vi "虚拟计算器_六控件查看.vi"() -> ()   [LabVIEW 2023]
doc: "实验1 简易计算器设计。按课程指导书建立六个字符串显示控件、初始化、While循环及数字、运算符、等号、清除值改变事件。四则运算条件结构直接位于等号事件内。"
panel:
  in  "清除":bool
  in  "等于":bool
  in  "除":bool
  in  "乘":bool
  in  "减":bool
  in  "加":bool
  in  "小数点":bool
  in  "数字0":bool
  in  "数字9":bool
  in  "数字8":bool
  in  "数字7":bool
  in  "数字6":bool
  in  "数字5":bool
  in  "数字4":bool
  in  "数字3":bool
  in  "数字2":bool
  in  "数字1":bool
  out "运算结果":string
  out "运算符临时值":string
  out "输入2":string
  out "输入1":string
  out "输入临时值":string
  out "过程显示":string
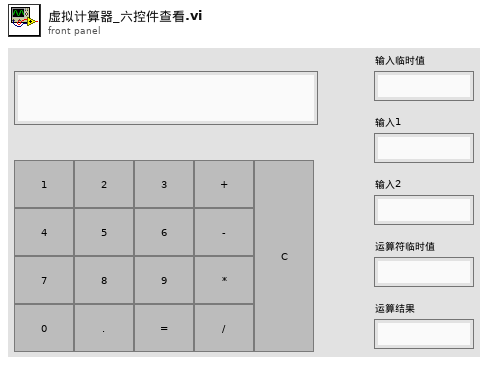
[diagram p1: front panel]
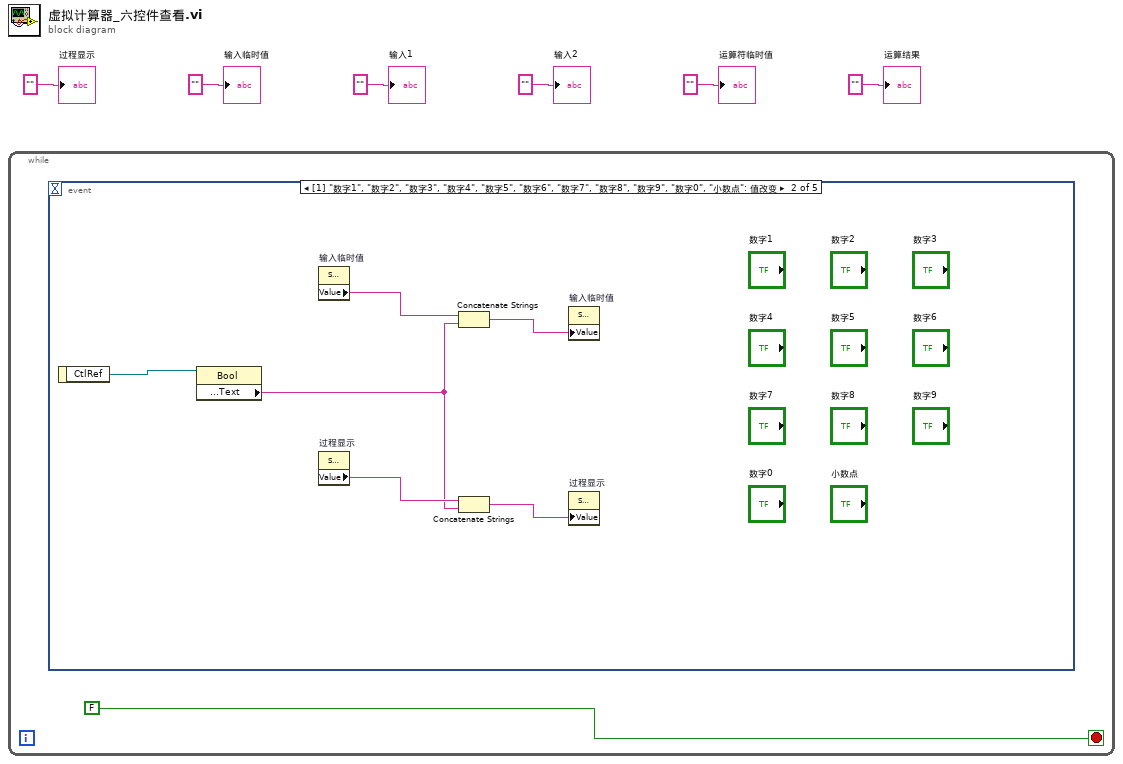
[diagram p0: block diagram]
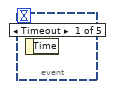
[diagram p2: hidden frame]
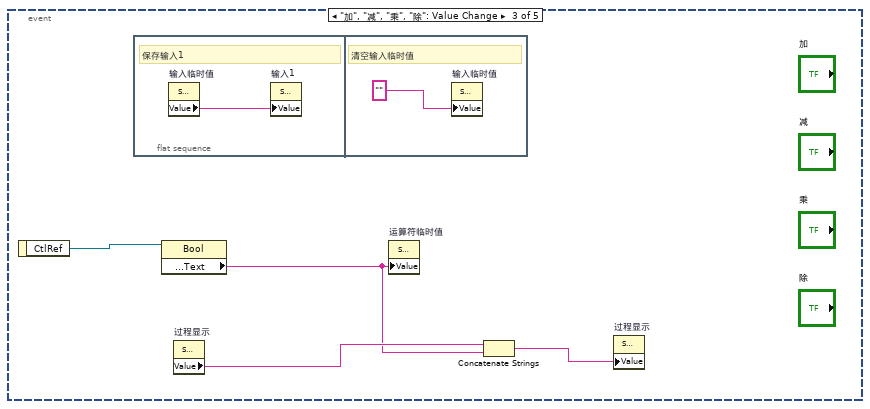
[diagram p3: hidden frame]
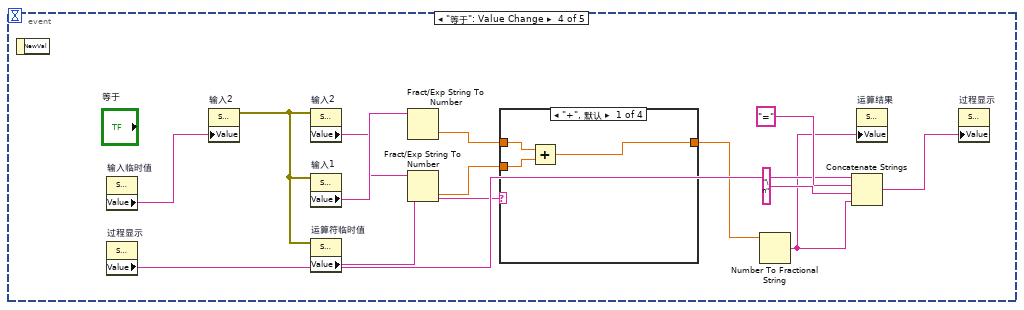
[diagram p4: hidden frame]
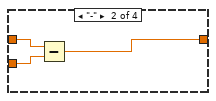
[diagram p5: hidden frame]
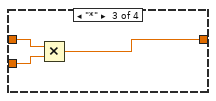
[diagram p6: hidden frame]
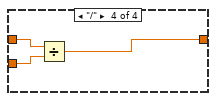
[diagram p7: hidden frame]
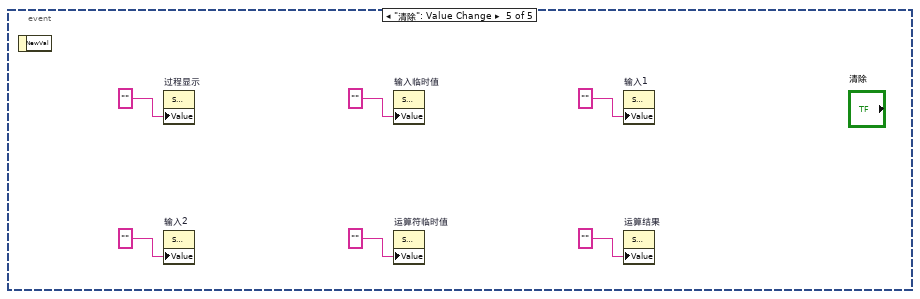
[diagram p8: hidden frame]
diagram:
  n1 = while {
    stop <- FALSE stop-if-true
    n2 = event shown="[1] \"数字1\", \"数字2\", \"数字3\", \"数字4\", \"数字5\", \"数字6\", \"数字7\", \"数字8\", \"数字9\", \"数字0\", \"小数点\": 值改变" {
      selector: _ -> [_ _ _ _ _]
      dyn-events: _ -> [_ _ _ _ _]
      timeout: _ -> [_ _ _ _ _]
      event Timeout {
        n3 = event-data() -> ()  [unwired: 1 in, 1 out]
      }
      event "数字1", "数字2", "数字3", "数字4", "数字5", "数字6", "数字7", "数字8", "数字9", "数字0", "小数点": Value Change {
        n4 = event-data() -> ("CtlRef"=w8:refnum<vi>)  [unwired: 1 in]
        n5 = property class="Bool"(reference=w8) -> ("Boolean Text.Text"=w9:string)  [unwired: 1 in, 2 out]
        n6 = property on="输入临时值" class="Str"() -> ("Value"=w10:string)  [unwired: 2 in, 2 out]
        n7 = property on="过程显示" class="Str"() -> ("Value"=w11:string)  [unwired: 2 in, 2 out]
        n8 = Concatenate Strings(w10, w9) -> (w12:string)
        n9 = Concatenate Strings(w11, w9) -> (w13:string)
        n10 = property on="输入临时值" class="Str"("Value"=w12) -> ()  [unwired: 2 in, 2 out]
        n11 = property on="过程显示" class="Str"("Value"=w13) -> ()  [unwired: 2 in, 2 out]
      }
      event "加", "减", "乘", "除": Value Change {
        n12 = event-data() -> ("CtlRef"=w14:refnum<vi>)  [unwired: 1 in]
        n13 = flat-sequence {
          frame #0 {
            # "保存输入1"
            n14 = property on="输入临时值" class="Str"() -> ("Value"=w18:string)  [unwired: 2 in, 2 out]
            n15 = property on="输入1" class="Str"("Value"=w18) -> ()  [unwired: 2 in, 2 out]
          }
          frame #1 {
            # "清空输入临时值"
            n16 = property on="输入临时值" class="Str"("Value"="") -> ()  [unwired: 2 in, 2 out]
          }
        }
        n17 = property class="Bool"(reference=w14) -> ("Boolean Text.Text"=w15:string)  [unwired: 1 in, 2 out]
        n18 = property on="过程显示" class="Str"() -> ("Value"=w16:string)  [unwired: 2 in, 2 out]
        n19 = property on="运算符临时值" class="Str"("Value"=w15) -> ()  [unwired: 2 in, 2 out]
        n20 = Concatenate Strings(w16, w15) -> (w17:string)
        n21 = property on="过程显示" class="Str"("Value"=w17) -> ()  [unwired: 2 in, 2 out]
      }
      event "等于": Value Change {
        n22 = event-data() -> ()  [unwired: 1 in, 1 out]
        n23 = property on="输入临时值" class="Str"() -> ("Value"=w20:string)  [unwired: 2 in, 2 out]
        n24 = property on="过程显示" class="Str"() -> ("Value"=w29:string)  [unwired: 2 in, 2 out]
        n25 = property on="输入2" class="Str"("Value"=w20) -> (error out=w21:errorcluster)  [unwired: 2 in, 1 out]
        n26 = property on="输入2" class="Str"(error in=w21) -> ("Value"=w22:string)  [unwired: 1 in, 2 out]
        n27 = property on="输入1" class="Str"(error in=w21) -> ("Value"=w23:string)  [unwired: 1 in, 2 out]
        n28 = property on="运算符临时值" class="Str"(error in=w21) -> ("Value"=w24:string)  [unwired: 1 in, 2 out]
        n29 = Fract/Exp String To Number(string=w23) -> (number=w25:dbl)  [unwired: 3 in, 1 out]
        n30 = Fract/Exp String To Number(string=w22) -> (number=w26:dbl)  [unwired: 3 in, 1 out]
        n31 = case shown="\"+\", 默认" w24 {
          tunnel: w25 -> [w33 w36 w39 w42]
          tunnel: w26 -> [w34 w37 w40 w43]
          tunnel: [w35 w38 w41 w44] -> w27
          frame "+", Default {
            n32 = Add(x=w33, y=w34) -> (x+y=w35:dbl)
          }
          frame "-" {
            n33 = Subtract(x=w36, y=w37) -> (x-y=w38:dbl)
          }
          frame "*" {
            n34 = Multiply(x=w39, y=w40) -> (x*y=w41:dbl)
          }
          frame "/" {
            n35 = Divide(x=w42, y=w43) -> (x/y=w44:dbl)
          }
        }
        n36 = Number To Fractional String(number=w27) -> (F-format string=w28:string)  [unwired: 3 out]
        n37 = Concatenate Strings(w29, "=", "\n", w28) -> (w32:string)
        n38 = property on="运算结果" class="Str"("Value"=w28) -> ()  [unwired: 2 in, 2 out]
        n39 = property on="过程显示" class="Str"("Value"=w32) -> ()  [unwired: 2 in, 2 out]
      }
      event "清除": Value Change {
        n40 = event-data() -> ()  [unwired: 1 in, 1 out]
        n41 = property on="过程显示" class="Str"("Value"="") -> ()  [unwired: 2 in, 2 out]
        n42 = property on="输入2" class="Str"("Value"="") -> ()  [unwired: 2 in, 2 out]
        n43 = property on="输入临时值" class="Str"("Value"="") -> ()  [unwired: 2 in, 2 out]
        n44 = property on="运算符临时值" class="Str"("Value"="") -> ()  [unwired: 2 in, 2 out]
        n45 = property on="输入1" class="Str"("Value"="") -> ()  [unwired: 2 in, 2 out]
        n46 = property on="运算结果" class="Str"("Value"="") -> ()  [unwired: 2 in, 2 out]
      }
    }
  }
  "过程显示" <- ""
  "输入临时值" <- ""
  "输入1" <- ""
  "输入2" <- ""
  "运算符临时值" <- ""
  "运算结果" <- ""
